vi "Write Stop Event.vi"(8 "error in":errorcluster, 10 "Stop Event":refnum<user-event>, 11 "Runner in":refnum<class "Runner.lvclass">) -> (0 "error out":errorcluster, 3 "Runner out":refnum<class "Runner.lvclass">)   [LabVIEW 2026, in "Runner.lvlib" / "Runner.lvclass"]
doc: "Data accessor."
uses:
  Runner.lvclass
  Runner.lvclass/Runner.ctl
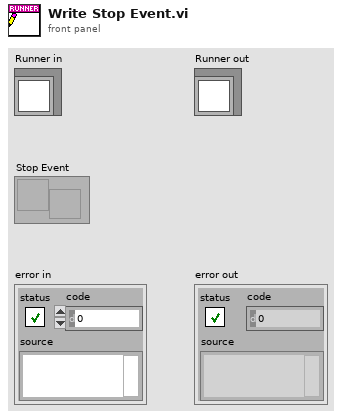
[diagram p1: front panel]
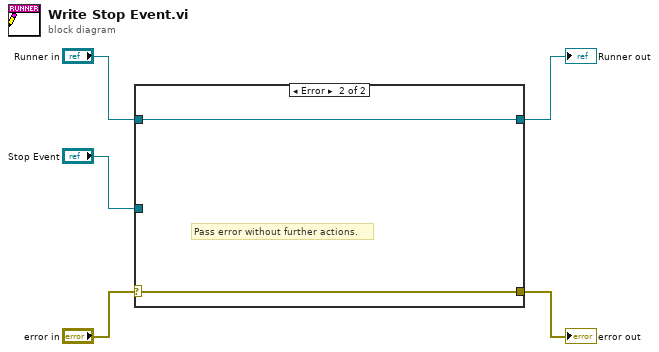
[diagram p0: block diagram]
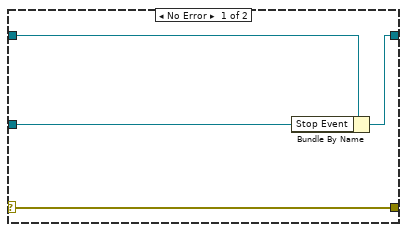
[diagram p2: hidden frame]
diagram:
  n1 = case shown="Error" "error in" {
    selector: "error in" -> [w9 w11]
    tunnel: [w9 w11] -> w4
    tunnel: [w7 w10] -> w2
    tunnel: "Runner in" -> [w8 w10]
    tunnel: "Stop Event" -> [w6 _]
    frame No Error {
      n2 = Bundle By Name(cluster=w8, "Stop Event"=w6) -> (w7:refnum<class "Runner.lvclass">)
    }
    frame Error {
      # "Pass error without further actions."
    }
  }
  "error out" <- w4
  "Runner out" <- w2
